vi "Set_Output.vi"(8 "error in (no error)":errorcluster, 10 "Output":dbl, 11 "object in":refnum<class "AIO_Channel.lvclass">) -> (0 "error out":errorcluster, 3 "object out":refnum<class "AIO_Channel.lvclass">)   [LabVIEW 2021, in "DAQmx.lvlib" / "AIO_Channel.lvclass"]
doc: "Sets the Digital Output"
uses:
  AIO_Channel.lvclass
  AIO_Channel.lvclass/AIO_Channel.ctl
  <vilib>/DAQmx/miscellaneous.llb/DAQmx Fill In Error Info.vi
  <vilib>/DAQmx/write.llb/DAQmx Write (Analog DBL 1Chan 1Samp).vi
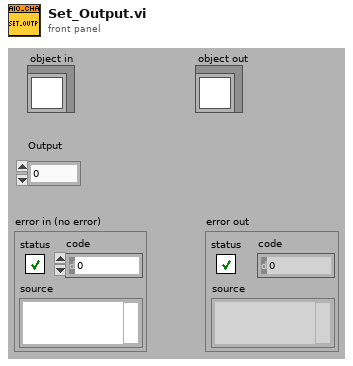
[diagram p1: front panel]
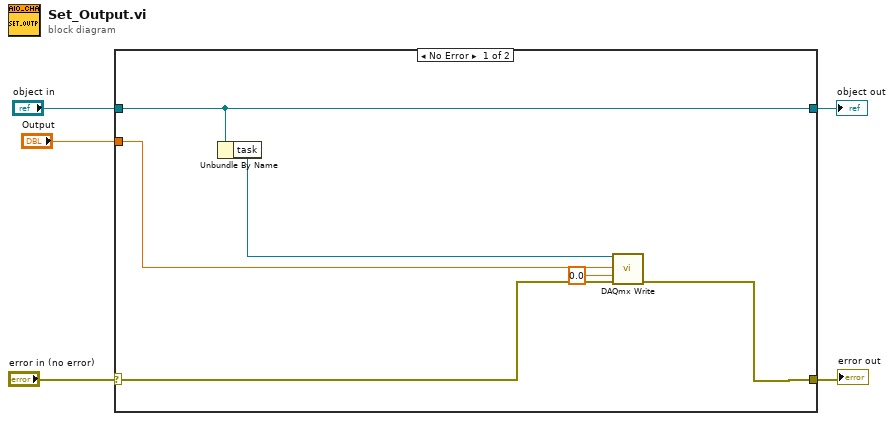
[diagram p0: block diagram]
diagram:
  n1 = case shown="No Error" "error in (no error)" {
    selector: "error in (no error)" -> [w8 w13]
    tunnel: [w7 w13] -> w4
    tunnel: [w11 w12] -> w2
    tunnel: "object in" -> [w11 w12]
    tunnel: "Output" -> [w6 _]
    frame No Error {
      n2 = Unbundle By Name(w11) -> ("task"=w9:refnum<k21>)
      n3 = call-poly <vilib>:"DAQmx Write.vi"("task/channels in"=w9, "data"=w6, "timeout"=0.0, "error in"=w8) -> ("error out"=w7:errorcluster)  [unwired: 9 in, 2 out]
    }
    frame Error {
    }
  }
  "error out" <- w4
  "object out" <- w2
